vi "Read Pixels and Copy to Display Image Array.vi"(0 "fpga interface in":refnum<k20>, 5 "display channel number":i32, 7 "serial channel display parameters":T4[](array[typedef]) {"RAW parameters"."bayer parameters"."blue gain" format="%_4g"; "RAW parameters"."bayer parameters"."green gain" format="%_4g"; "RAW parameters"."bayer parameters"."red gain" format="%_4g"; "RAW parameters"."bayer parameters"."algorithm" items=["Bilinear", "VNG"]; "RAW parameters"."bayer parameters"."pattern" items=["GB", "GR", "BG", "RG"]}, 9 "image metadata":T2, 11 "error in (no error)":errorcluster) -> (4 "fpga interface out":refnum<k20>, 6 "display image":T1, 8 "Pixel Data":u32[](array[numeric]), 15 "error out":errorcluster)   [LabVIEW 2025, in "Automotive Vision.lvclass"]
uses:
  Automotive Vision.lvclass
  Automotive Vision.lvclass/Automotive Vision.ctl
  deps/NI148X/Getting Started/Host/Common/GettingStarted_Common_148X_Host.lvlib
  <instrlib>/FlexRIO/CSI-2/v2/Common/Types/LLP Data Type.ctl
  <instrlib>/FlexRIO/CSI-2/v2/Common/NI CSI-2 API Common v2.lvlib
  <vilib>/vision/Image Controls.llb/IMAQ Image.ctl
  deps/NI148X/Getting Started/Host/Common/Types/Serial Channel Display Parameters.ctl
  deps/NI148X/Getting Started/FPGA/Common/Types/Image Metadata.ctl
  deps/NI148X/Getting Started/FPGA/Common/GettingStarted_Common_148X_FPGA.lvlib
  deps/NI148X/Getting Started/Host/Common/Types/RAW Interpretation for Display.ctl
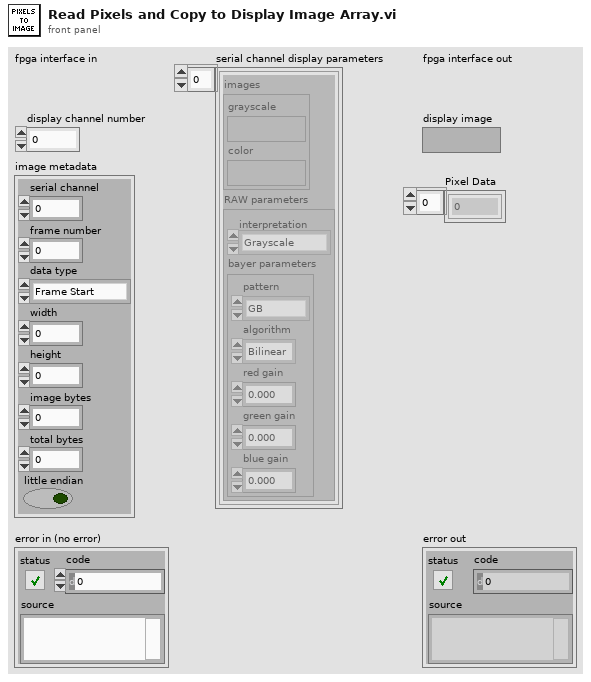
[diagram p1: front panel]
types:
  T1 = typedef "IMAQ Image.ctl" = refnum<image>
  T2 = typedef "GettingStarted_Common_148X_FPGA.lvlib/Image Metadata.ctl" = cluster{"serial channel":fxp<+,3,3>, "frame number":u16, "data type":T3, "width":u16, "height":u16, "image bytes":u32, "total bytes":u32, "little endian":bool}
  T3 = typedef "NI CSI-2 API Common v2.lvlib/LLP Data Type.ctl" = enum8{"Frame Start", "Frame End", "Line Start", "Line End", "End of Transmission", "Reserved 0", "Reserved 1", "Reserved 2", "Generic Short Packet 1", "Generic Short Packet 2", "Generic Short Packet 3", "Generic Short Packet 4", "Generic Short Packet 5", "Generic Short Packet 6", "Generic Short Packet 7", "Generic Short Packet 8", "Null", "Blanking Data", "Embedded 8-bit non Image Data", "Generic Long Packet 1", "Generic Long Packet 2", "Generic Long Packet 3", "Generic Long Packet 4", "Reserved 3", "YUV420 8-bit", "YUV420 10-bit", "Legacy YUV420 8-bit", "Reserved 4", "YUV420 8-bit Chroma Shifted", "YUV420 10-bit Chroma Shifted", "YUV422 8-bit", "YUV422 10-bit", "RGB444", "RGB555", "RGB565", "RGB666", "RGB888", "Reserved 5", "Reserved 6", "RAW 24", "RAW 6", "RAW 7", "RAW 8", "RAW 10", "RAW 12", "RAW 14", "RAW 16", "RAW 20", "User Defined 8-bit Data 1", "User Defined 8-bit Data 2", "User Defined 8-bit Data 3", "User Defined 8-bit Data 4", "User Defined 8-bit Data 5", "User Defined 8-bit Data 6", "User Defined 8-bit Data 7", "User Defined 8-bit Data 8", "USL Command", "Reserved 7", "Reserved 8", "Reserved 9", "Reserved 10", "Reserved 11", "Reserved 12", "LRTE EPD Spacer"}
  T4 = typedef "GettingStarted_Common_148X_Host.lvlib/Serial Channel Display Parameters.ctl" = cluster{"images":cluster{"grayscale":T1, "color":T1}, "RAW parameters":cluster{"interpretation":T5, "bayer parameters":cluster{"pattern":i32, "algorithm":i32, "red gain":dbl, "green gain":dbl, "blue gain":dbl}}}
  T5 = typedef "GettingStarted_Common_148X_Host.lvlib/RAW Interpretation for Display.ctl" = enum16{"Grayscale", "Bayer", "RGB", "YUV422", "YUV420", "Legacy YUV420"}
  T6 = cluster{"pattern":i32, "algorithm":i32, "red gain":dbl, "green gain":dbl, "blue gain":dbl}
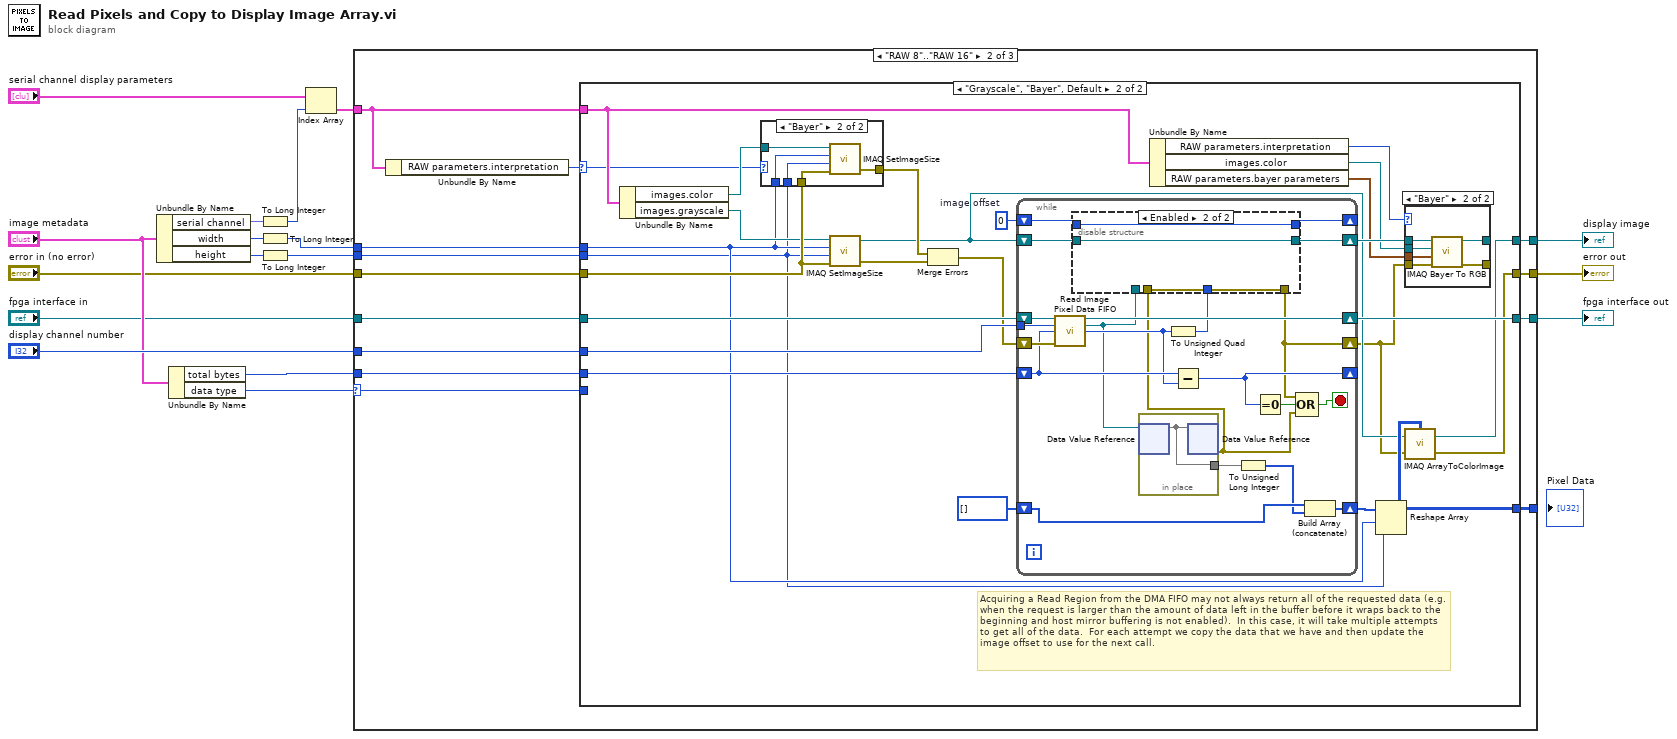
[diagram p0: block diagram]
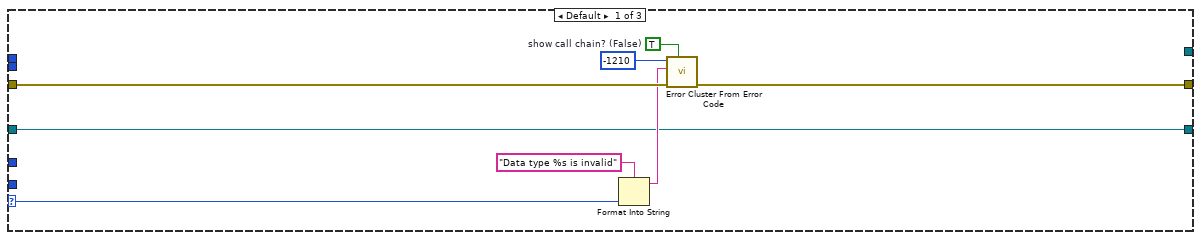
[diagram p2: hidden frame]
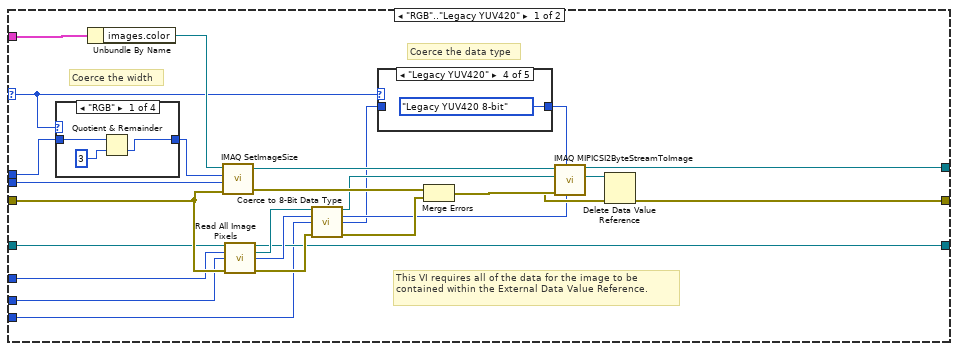
[diagram p3: hidden frame]
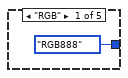
[diagram p4: hidden frame]
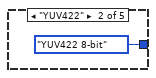
[diagram p5: hidden frame]
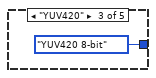
[diagram p6: hidden frame]
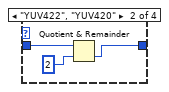
[diagram p8: hidden frame]
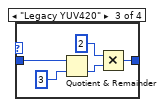
[diagram p9: hidden frame]
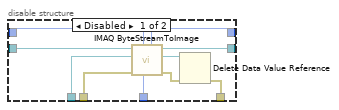
[diagram p12: hidden frame]
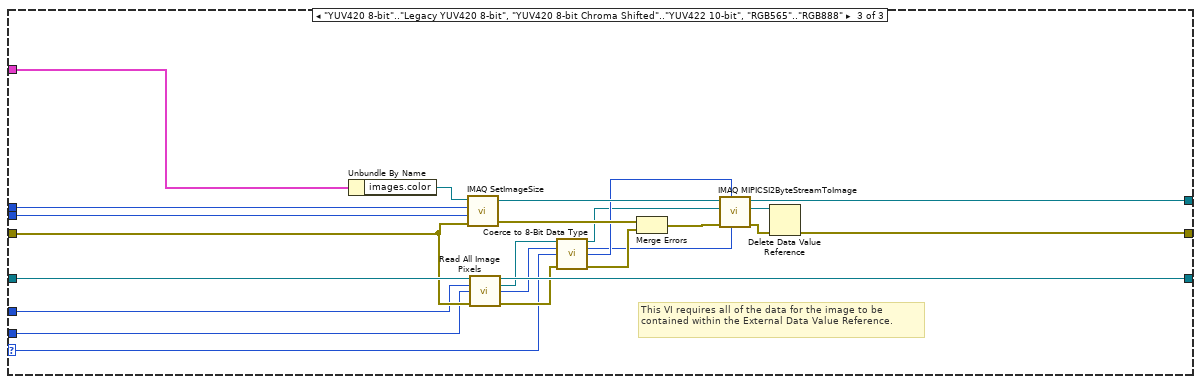
[diagram p14: hidden frame]
diagram:
  n1 = Unbundle By Name("image metadata") -> ("serial channel"=w13:fxp<+,3,3>, "width"=w9:u16, "height"=w10:u16)
  n2 = Unbundle By Name("image metadata") -> ("total bytes"=w16:u32, "data type"=w1:T3)
  n3 = To Long Integer(number=w13) -> (32bit integer=w11:i32)
  n4 = To Long Integer(number=w9) -> (32bit integer=w6:i32)
  n5 = To Long Integer(number=w10) -> (32bit integer=w7:i32)
  n6 = Index Array(array="serial channel display parameters", index=w11) -> (element=w3:T4)
  n7 = case shown="\"RAW 8\"..\"RAW 16\"" w1 {
    selector: w1 -> [w19 w27 w161]
    tunnel: w16 -> [_ w38 w171]
    tunnel: [w18 w37 w173] -> w15
    tunnel: "display channel number" -> [_ w36 w170]
    tunnel: "error in (no error)" -> [w23 w35 w174]
    tunnel: w7 -> [_ w34 w181]
    tunnel: w6 -> [_ w33 w180]
    tunnel: [_ w32 w169] -> w5
    tunnel: [w22 w31 w166] -> w4
    tunnel: w3 -> [_ w29 w178]
    tunnel: "fpga interface in" -> [w18 w30 w177]
    tunnel: [_ w26 _] -> _
    frame Default {
      w24 = TRUE  # show call chain? (False)
      n8 = Format Into String(format string="Data type %s is invalid" ("error message (\"\")"), w19) -> (resulting string=w20:string)  [unwired: 2 in, 1 out]
      n9 = call <vilib>:"Error Cluster From Error Code.vi"("show call chain? (False)"=w24, "error in (no error)"=w23, "error message (\"\")"=w20, "error code (0)"=-1210) -> ("error out"=w22:errorcluster)  [unwired: 5 in]
    }
    frame "RAW 8".."RAW 16" {
      n10 = Unbundle By Name(w29) -> ("RAW parameters.interpretation"=w28:T5)
      n11 = case shown="\"Grayscale\", \"Bayer\", Default" w28 {
        selector: w28 -> [w41 w93]
        tunnel: w38 -> [w48 w108]
        tunnel: [w52 w106] -> w37
        tunnel: w36 -> [w47 w105]
        tunnel: w35 -> [w53 w104]
        tunnel: w34 -> [w44 w87]
        tunnel: w33 -> [w43 w88]
        tunnel: [w50 w86] -> w32
        tunnel: [w51 w83] -> w31
        tunnel: w29 -> [w46 w97]
        tunnel: w30 -> [w49 w96]
        tunnel: w27 -> [w45 _]
        tunnel: [_ w89] -> w26
        frame "RGB".."Legacy YUV420" {
          # "Coerce the data type"
          # "Coerce the width"
          # "This VI requires all of the data for the image to be contained within the External Data Value Reference."
          n12 = case shown="\"RGB\"" w41 {
            tunnel: w43 -> [w72 w75 w81 w82]
            tunnel: [w71 w74 w78 w82] -> w42
            frame "RGB" {
              n13 = Quotient & Remainder(x=w72, y=3) -> (floor(x/y)=w71:i32)  [unwired: 1 out]
            }
            frame "YUV422", "YUV420" {
              n14 = Quotient & Remainder(x=w75, y=2) -> (floor(x/y)=w74:i32)  [unwired: 1 out]
            }
            frame "Legacy YUV420" {
              n15 = Quotient & Remainder(x=w81, y=3) -> (floor(x/y)=w79:i32)  [unwired: 1 out]
              n16 = Multiply(x=2, y=w79) -> (x*y=w78:i32)
            }
            frame Default {
            }
          }
          n17 = Unbundle By Name(w46) -> ("images.color"=w65:T1)
          n18 = call "IMAQ SetImageSize"("error in (no error)"=w53, "Y Resolution"=w44, "X Resolution"=w42, "Image"=w65) -> ("error out"=w63:errorcluster, "Image Out"=w64:T1)  [unwired: 1 in]
          n19 = call "Read All Image Pixels.vi"("fpga inteface in"=w49, "display channel number"=w47, "image bytes"=w48, "error in (no error)"=w53) -> ("fpga interface out"=w52:refnum<k20>, "image pixel data region"=w58:refnum<data-value>, "elements in region"=w57:u32, "error out"=w59:errorcluster)  [unwired: 8 in]
          n20 = call "Coerce to 8-Bit Data Type.vi"("image pixel data region in"=w58, "image bytes in"=w57, "data type in"=w45, "error in (no error)"=w59) -> ("image pixel data region out"=w54:refnum<data-value>, "image bytes out"=w55:u32, "data type out"=w39:T3, "error out"=w56:errorcluster)  [unwired: 8 in]
          n21 = case shown="\"Legacy YUV420\"" w41 {
            tunnel: w39 -> [_ _ _ _ w70]
            tunnel: [LLP_Data_Type."RGB888" ("data type") LLP_Data_Type."YUV422 8-bit" ("data type") LLP_Data_Type."YUV420 8-bit" ("data type") LLP_Data_Type."Legacy YUV420 8-bit" ("data type") w70] -> w40
            frame "RGB" {
            }
            frame "YUV422" {
            }
            frame "YUV420" {
            }
            frame "Legacy YUV420" {
            }
            frame Default {
            }
          }
          n22 = Merge Errors(w63, w56) -> (w62:errorcluster)
          n23 = call "IMAQ MIPICSI2ByteStreamToImage"("Bytes to Copy"=w55, "Format"=w40, "error in (no error)"=w62, "Byte Stream In"=w54, "Image In"=w64) -> ("error out"=w61:errorcluster, "Byte Stream Out"=w60:refnum<data-value>, "Image Out"=w50:T1)  [unwired: 3 in, 1 out]
          n24 = Delete Data Value Reference(data value reference=w60, error in=w61) -> (error out=w51:errorcluster)  [unwired: 1 out]
        }
        frame "Grayscale", "Bayer", Default {
          w94 = u32 0  # image offset
          # "Acquiring a Read Region from the DMA FIFO may not always return all of the requested data (e.g. when the request is larger than the amount of data left in the buffer before it wraps back to the beginning and host mirror buffering is not enabled).  In this case, it will take multiple attempts to get all of the data.  For each attempt we copy the data that we have and then update the image offset to use for the next call."
          n25 = Unbundle By Name(w97) -> ("images.color"=w102:T1, "images.grayscale"=w90:T1)
          n26 = case shown="\"Bayer\"" w93 {
            tunnel: w104 -> [w109 w114]
            tunnel: [w109 w113] -> w103
            tunnel: w102 -> [_ w112]
            tunnel: w87 -> [_ w111]
            tunnel: w88 -> [_ w110]
            frame "Grayscale", Default {
            }
            frame "Bayer" {
              n27 = call "IMAQ SetImageSize"("error in (no error)"=w114, "Y Resolution"=w111, "X Resolution"=w110, "Image"=w112) -> ("error out"=w113:errorcluster)  [unwired: 1 in, 1 out]
            }
          }
          n28 = call "IMAQ SetImageSize"("error in (no error)"=w104, "Y Resolution"=w87, "X Resolution"=w88, "Image"=w90) -> ("error out"=w107:errorcluster, "Image Out"=w85:T1)  [unwired: 1 in]
          n29 = Merge Errors(w103, w107) -> (w95:errorcluster)
          n30 = while {
            tunnel: w105 -> [w133]
            shift-right: [w134] -> w106
            shift-left: w96 -> [w135]
            shift-right: [w123] -> w84
            shift-left: w95 -> [w132]
            shift-right: [w130] -> w101
            shift-left: w85 -> [w131]
            shift-right: [w126] -> _
            shift-left: w108 -> [w128]
            shift-right: [w122] -> _
            shift-left: w94 -> [w121]
            shift-right: [w119] -> w91
            shift-left: u32[] [] -> [w118]
            stop <- w124 stop-if-true
            n31 = call "Read Image Pixel Data FIFO.vi"("fpga inteface in"=w135, "display channel number"=w133, "number of elements"=w128, "error in (no error)"=w132) -> ("fpga interface out"=w134:refnum<k20>, "image pixel data region"=w117:refnum<data-value>, "elements in region"=w127:u32)  [unwired: 7 in, 2 out]
            n32 = in-place {
              in-place-border: [w149] -> w120
              n33 = in-place-dvr #1(w117) -> (w149:u8[])  [unwired: 1 out]
              n34 = in-place-dvr #1(w149) -> (w116:errorcluster)  [unwired: 1 out]
            }
            n35 = To Unsigned Quad Integer(1:w127) -> (0:w129:u64)
            n36 = disable-structure shown="Enabled" {
              disable-tunnel: w131 -> [w145 w148]
              disable-tunnel: [w144 w148] -> w130
              disable-tunnel: w116 -> [w143 w147]
              disable-tunnel: w129 -> [w142 _]
              disable-tunnel: [w139 w147] -> w123
              disable-tunnel: [w138 w146] -> w122
              disable-tunnel: w121 -> [w137 w146]
              disable-tunnel: w117 -> [w136 _]
              frame Disabled {
                n37 = call "IMAQ ByteStreamToImage"("Bytes to Copy"=w142, "Image Byte Offset In"=w137, "error in (no error)"=w143, "Byte Stream In"=w136, "Image In"=w145) -> ("error out"=w140:errorcluster, "Byte Stream Out"=w141:refnum<data-value>, "Image Out"=w144:T1, "Image Byte Offset Out"=w138:u32)  [unwired: 2 in, 1 out]
                n38 = Delete Data Value Reference(data value reference=w141, error in=w140) -> (error out=w139:errorcluster)  [unwired: 1 out]
              }
              frame Enabled {
              }
            }
            n39 = Subtract(x=w128, y=w127) -> (x-y=w126:u32)
            n40 = To Unsigned Long Integer(number=w120) -> (unsigned 32bit integer=w115:u32[])
            n41 = Equal To 0?(x=w126) -> (x = 0?=w125:bool)
            n42 = Compound Arithmetic op=OR(w123, w125, w116) -> (w124:bool)
            n43 = Build Array (concatenate)(w118, w115) -> (w119:u32[])
          }
          n44 = Unbundle By Name(w97) -> ("RAW parameters.interpretation"=w98:T5, "images.color"=w99:T1, "RAW parameters.bayer parameters"=w100:T6)
          n45 = Reshape Array(w91, w88, w87) -> (w89:u32[][])
          n46 = case shown="\"Bayer\"" w98 {
            tunnel: w101 -> [w150 w157]
            tunnel: [w150 w156] -> _
            tunnel: w84 -> [w151 w155]
            tunnel: [w151 w154] -> _
            tunnel: w99 -> [_ w153]
            tunnel: w100 -> [_ w152]
            frame "Grayscale", Default {
            }
            frame "Bayer" {
              n47 = call "IMAQ Bayer To RGB"("error in (no error)"=w155, "Bayer Parameters"=w152, "Image Dst"=w153, "Image Src"=w157) -> ("error out"=w154:errorcluster, "Image Dst Out"=w156:T1)  [unwired: 6 in]
            }
          }
          n48 = call "IMAQ ArrayToColorImage"("Image Pixels (U32)"=w89, "Image"=w85, "error in (no error)"=w84) -> ("Image Out"=w86:T1, "error out"=w83:errorcluster)  [unwired: 2 in]
        }
      }
    }
    frame "YUV420 8-bit".."Legacy YUV420 8-bit", "YUV420 8-bit Chroma Shifted".."YUV422 10-bit", "RGB565".."RGB888" {
      # "This VI requires all of the data for the image to be contained within the External Data Value Reference."
      n49 = Unbundle By Name(w178) -> ("images.color"=w179:T1)
      n50 = call "IMAQ SetImageSize"("error in (no error)"=w174, "Y Resolution"=w181, "X Resolution"=w180, "Image"=w179) -> ("error out"=w175:errorcluster, "Image Out"=w176:T1)  [unwired: 1 in]
      n51 = call "Read All Image Pixels.vi"("fpga inteface in"=w177, "display channel number"=w170, "image bytes"=w171, "error in (no error)"=w174) -> ("fpga interface out"=w173:refnum<k20>, "image pixel data region"=w164:refnum<data-value>, "elements in region"=w163:u32, "error out"=w165:errorcluster)  [unwired: 8 in]
      n52 = call "Coerce to 8-Bit Data Type.vi"("image pixel data region in"=w164, "image bytes in"=w163, "data type in"=w161, "error in (no error)"=w165) -> ("image pixel data region out"=w158:refnum<data-value>, "image bytes out"=w159:u32, "data type out"=w160:T3, "error out"=w162:errorcluster)  [unwired: 8 in]
      n53 = Merge Errors(w175, w162) -> (w172:errorcluster)
      n54 = call "IMAQ MIPICSI2ByteStreamToImage"("Bytes to Copy"=w159, "Format"=w160, "error in (no error)"=w172, "Byte Stream In"=w158, "Image In"=w176) -> ("error out"=w168:errorcluster, "Byte Stream Out"=w167:refnum<data-value>, "Image Out"=w169:T1)  [unwired: 3 in, 1 out]
      n55 = Delete Data Value Reference(data value reference=w167, error in=w168) -> (error out=w166:errorcluster)  [unwired: 1 out]
    }
  }
  "display image" <- w5
  "fpga interface out" <- w15
  "error out" <- w4
